vi "GV-GraphHoverAddYaxis.vi"(8 "error in (no error)":errorcluster, 9 "Coords":T1, 11 "Gviewer in":refnum<class "Gviewer.lvclass">) -> (0 "error out":errorcluster, 1 "Plot Images:Front":picture, 3 "Gviewer out":refnum<class "Gviewer.lvclass">)   [LabVIEW 2020, in "Sgraph_lib_V1.lvlib" / "Gviewer.lvclass"]
doc: "Andre Koelewijn, 27 April 2021\n\nMove legend over the graph area"
uses:
  Gviewer.lvclass
  <vilib>/Utility/miscctls.llb/LVPoint32TypeDef.ctl
  Gviewer.lvclass/Gviewer.ctl
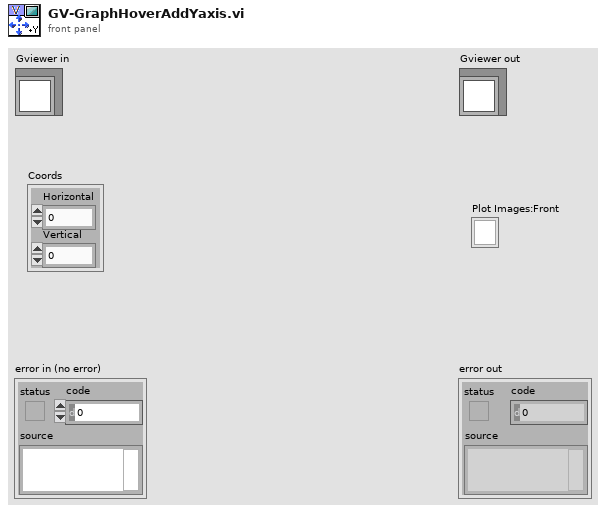
[diagram p1: front panel]
types:
  T1 = typedef "LVPoint32TypeDef.ctl" = cluster{"Horizontal":i32, "Vertical":i32}
  T2 = typedef "LVPositionTypeDef.ctl" = cluster{"Left":i32, "Top":i32}
  T3 = typedef "LVRectTypeDef.ctl" = cluster{"Left":i16, "Top":i16, "Right":i16, "Bottom":i16}
  T4 = typedef "LVBoundsTypeDef.ctl" = cluster{"Width":u32, "Height":u32}
  T5 = typedef "Sgraph_lib_V1.lvlib/Gviewer.lvclass/LegendSet.ctl" = cluster{"Position":T2, "Size":T4, "Rows":u32, "Select":i32, "Visible":bool}
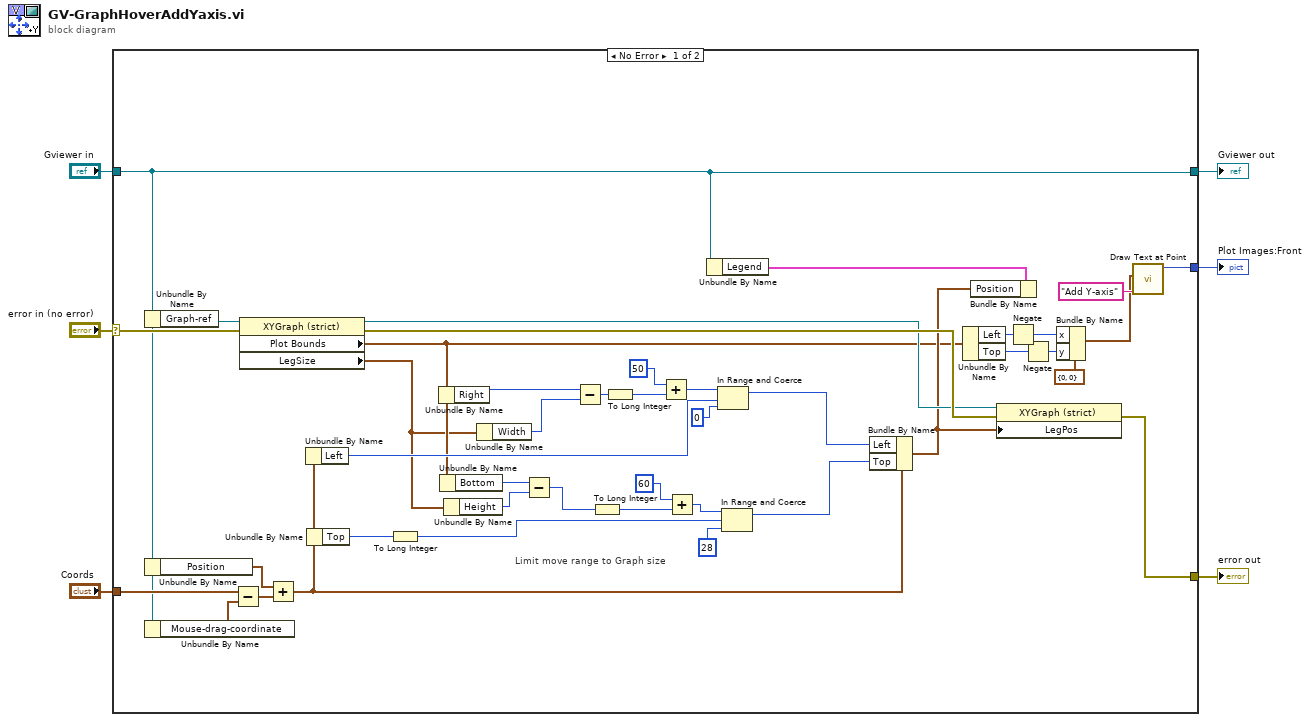
[diagram p0: block diagram]
diagram:
  n1 = case shown="No Error" "error in (no error)" {
    selector: "error in (no error)" -> [w37 w50]
    tunnel: [w35 w50] -> w5
    tunnel: [w33 w49] -> w3
    tunnel: "Gviewer in" -> [w33 w49]
    tunnel: "Coords" -> [w36 _]
    tunnel: [w9 _] -> w1
    frame No Error {
      # "Limit move range to Graph size"
      n2 = Unbundle By Name(w33) -> ("Graph-ref"=w39:refnum<vi>)
      n3 = Unbundle By Name(w33) -> ("Position"=w47:T2)
      n4 = Unbundle By Name(w33) -> ("Mouse-drag-coordinate"=w48:T1)
      n5 = Subtract(x=w36, y=w48) -> (x-y=w46:T1)
      n6 = property class="XYGraph (strict)"(reference=w39, error in=w37) -> (reference out=w34:refnum<vi>, error out=w40:errorcluster, "Plot Bounds"=w18:T3, "LegSize"=w15:T4)
      n7 = Add(x=w47, y=w46) -> (x+y=w22:T2)
      n8 = Unbundle By Name(w22) -> ("Left"=w29:i32)
      n9 = Unbundle By Name(w22) -> ("Top"=w20:i32)
      n10 = To Long Integer(number=w20) -> (32bit integer=w11:i32)
      n11 = Unbundle By Name(w18) -> ("Right"=w27:i16)
      n12 = Unbundle By Name(w18) -> ("Bottom"=w17:i16)
      n13 = Unbundle By Name(w15) -> ("Height"=w16:u32)
      n14 = Unbundle By Name(w15) -> ("Width"=w30:u32)
      n15 = Subtract(x=w17, y=w16) -> (x-y=w13:u32)
      n16 = Subtract(x=w27, y=w30) -> (x-y=w26:u32)
      n17 = To Long Integer(number=w13) -> (32bit integer=w10:i32)
      n18 = To Long Integer(number=w26) -> (32bit integer=w25:i32)
      n19 = Add(x=50, y=w25) -> (x+y=w23:i32)
      n20 = Add(x=60, y=w10) -> (x+y=w12:i32)
      n21 = Unbundle By Name(w33) -> ("Legend"=w38:T5)
      n22 = In Range and Coerce(upper limit=w23, x=w29, lower limit=0) -> (coerced(x)=w31:i32)  [unwired: 1 out]
      n23 = In Range and Coerce(upper limit=w12, x=w11, lower limit=28) -> (coerced(x)=w21:i32)  [unwired: 1 out]
      n24 = Bundle By Name(cluster=w22, "Left"=w31, "Top"=w21) -> (w32:T2)
      n25 = Unbundle By Name(w18) -> ("Left"=w42:i16, "Top"=w44:i16)
      n26 = Bundle By Name(cluster=w38, "Position"=w32) -> ()  [unwired: 1 out]
      n27 = property class="XYGraph (strict)"(reference=w34, error in=w40, "LegPos"=w32) -> (error out=w35:errorcluster)  [unwired: 1 out]
      n28 = Negate(x=w42) -> (-x=w43:i16)
      n29 = Negate(x=w44) -> (-x=w45:i16)
      n30 = Bundle By Name(cluster=cluster{"x":i16, "y":i16} {"x"=0, "y"=0}, "x"=w43, "y"=w45) -> (w7:cluster{"x":i16, "y":i16})
      n31 = call <vilib>:"Draw Text at Point.vi"("text"="Add Y-axis", "origin"=w7) -> ("new picture"=w9:picture)  [unwired: 8 in, 1 out]
    }
    frame Error {
    }
  }
  "error out" <- w5
  "Gviewer out" <- w3
  "Plot Images:Front" <- w1
